vi "VIH Dialog - Compiled HTML Help  Project.vi"(11 "Project Tree":T1) -> ()   [LabVIEW 2014]
doc: "::: VI Helpeks :::\nCopyright (c) 2000-2026 Konstantin Shifershteyn. All rights reserved."
uses:
  VIH Project Tree Typedef - Tree Refnum.ctl
  <vilib>/Platform/browser.llb/Open URL in Default Browser (string).vi
  <vilib>/Platform/browser.llb/Open URL in Default Browser (path).vi
panel:
  in  "Tab Control":enum32{"Project", "Options", "Compile Log"}(tab)
  in  "%HHP New Compile":bool caption="Create & Compile"
  in  "%HHP Info":bool caption="Open Info File"
  in  "%HHP Open":bool caption="Open Project"
  in  "%CHM Open":bool caption="Open CHM File"
  in  "HHP Target Path":path caption="HHP File"
  in  "HHP Target":enum16{"default", "custom"}(ring) caption="Default/Custom selector"
  in  "Default Topic Path":path caption="Default Topic File"
  in  "Default Topic":enum16{"auto", "custom"}(ring) caption="Auto/Custom selector"
  in  "%HHP Explore":bool caption="Explore Folder"
  in  "CHM File Path":path caption="CHM File"
  in  "Custom CHM":enum16{"default", "custom"}(ring) caption="Default/Custom selector"
  in  "Create IDX file":bool=TRUE caption="Generate Index file (HHK)"
  in  "Create TOC file":bool=TRUE caption="Generate Contents file (HHC)"
  in  "%HHP Create":bool caption="Create Project"
  in  "%CHM Compile":bool caption="Create & Compile"
  in  "CHM_AutoBuild":bool caption="Compile CHM file after HTML files are built (HHP file must exist)"
  in  "HHP_AutoBuild":bool caption="Generate HHP file after HTML files are built"
  in  "Open CHM After Compiling":bool=TRUE caption="Open CHM file after compiling"
  in  "HHP Template Path":path caption="HHP Template File"
  in  "HHP Template":enum16{"default", "custom"}(ring) caption="Default/Custom selector"
  in  "OpenAfterBuild":bool=TRUE caption="Open HTML Help Project file (HHP) after creation"
  out "CompileLog":string caption="Compile Log"
  in  "Cancel":bool
  # "*) use Context Help for information on the controls"
  # "HTML Help Project (HHP)"
  # "Compiled Help File (CHM)"
  # "Default Topic (HTML File)"
  # "HHP Template File"
  # "Options used in this utility"
  # "Options used when build from main window"
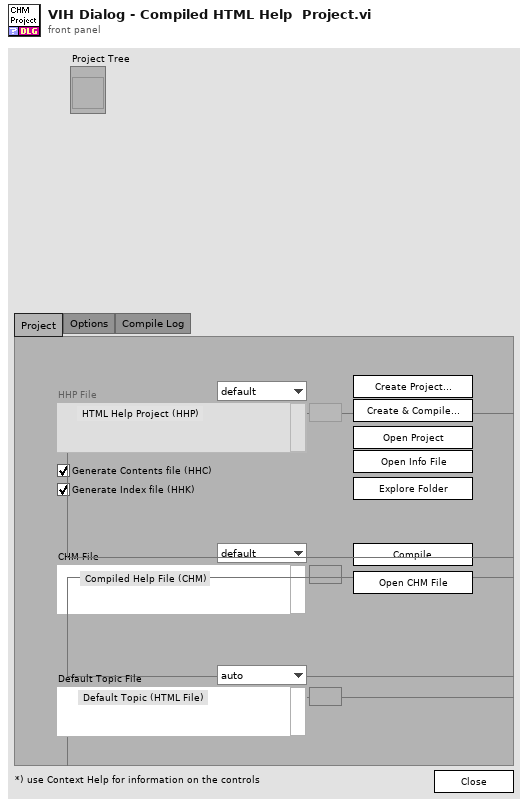
[diagram p1: front panel]
types:
  T1 = typedef "VIH Project Tree Typedef - Tree Refnum.ctl" = refnum<vi>
  T2 = typedef "VIH - CHM Project - HHP Generation Params Cluster.ctl" = cluster{"HHP_Template":enum16{"default", "custom"}, "HHP_Template_CustomPath":path, "HHP_Target":enum16{"default", "custom"}, "HHP_Target_CustomPath":path, "HHP_CreateTOC":bool, "HHP_CreateIDX":bool, "HHP_DefaultTopic":enum16{"auto", "custom"}, "HHP_DefaultTopic_CustomPath":path, "CHM_Filename":path, "HHP_AutoBuild":bool, "CHM_AutoBuild":bool}
  T3 = cluster{"Windows platform":bool, "HHP is associated":bool, "HHC is installed":bool}
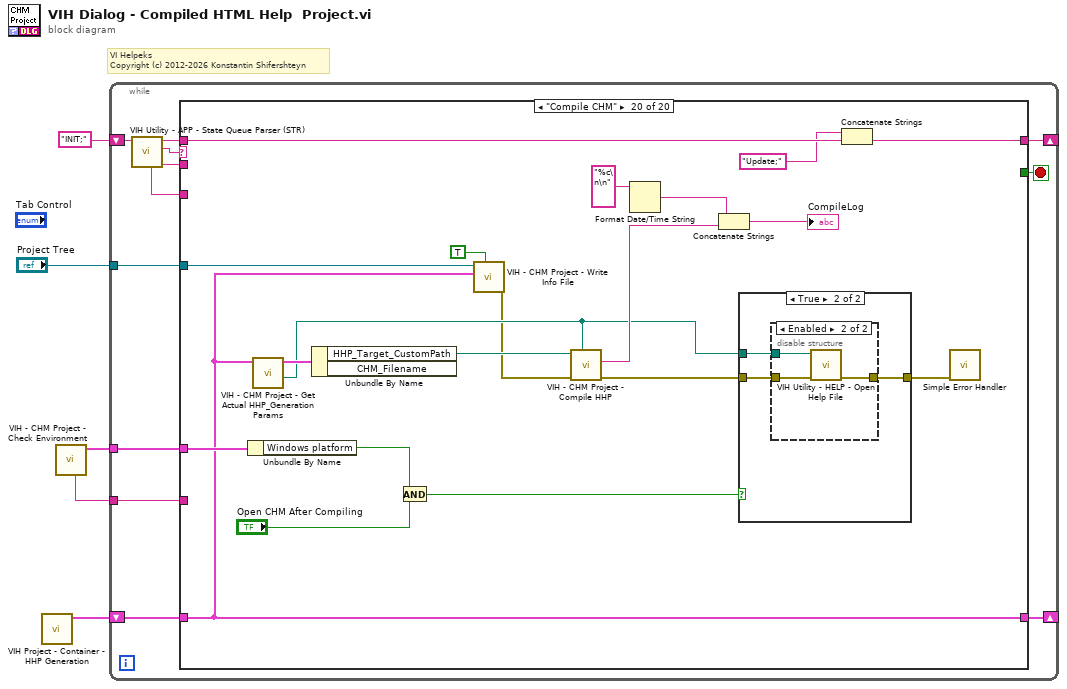
[diagram p0: block diagram]
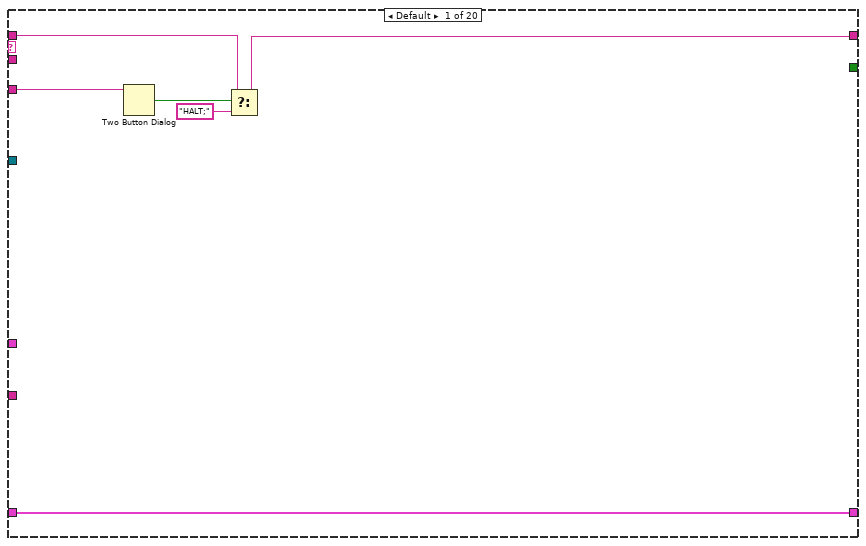
[diagram p2: hidden frame]
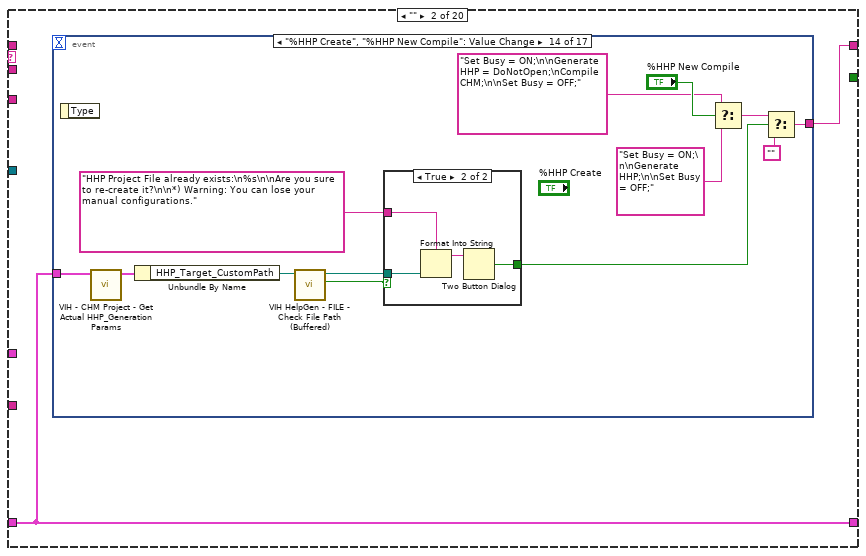
[diagram p3: hidden frame]
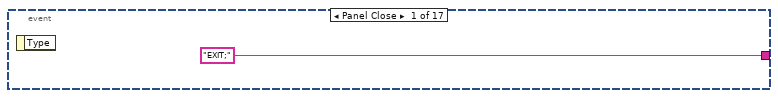
[diagram p4: hidden frame]
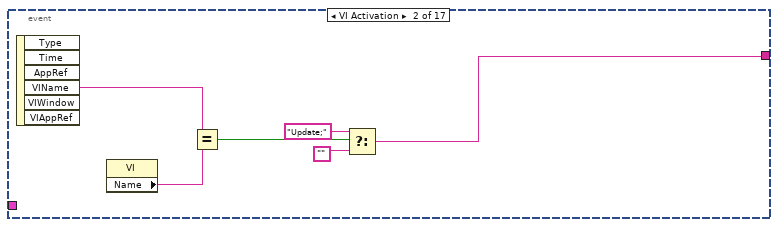
[diagram p5: hidden frame]
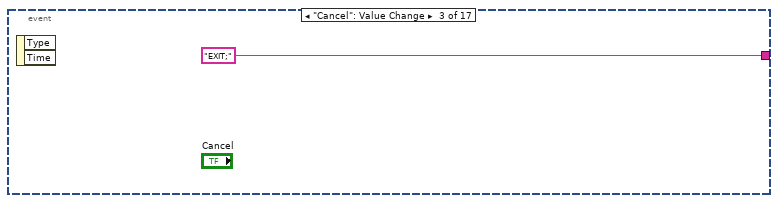
[diagram p6: hidden frame]
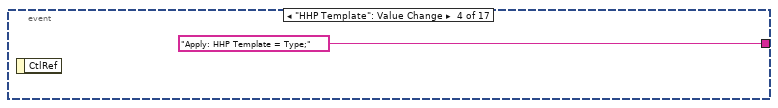
[diagram p7: hidden frame]
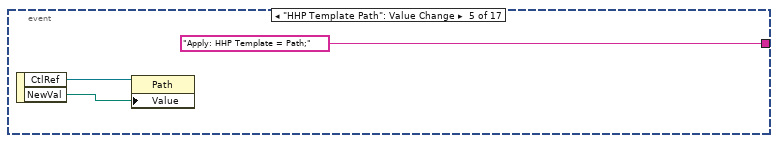
[diagram p8: hidden frame]
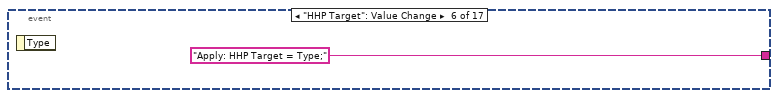
[diagram p9: hidden frame]
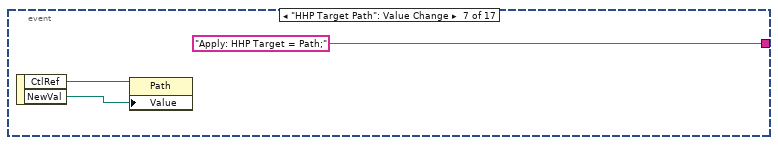
[diagram p10: hidden frame]
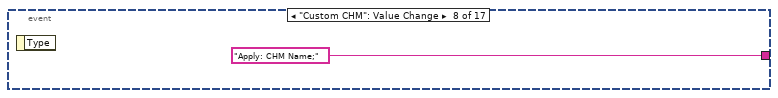
[diagram p11: hidden frame]
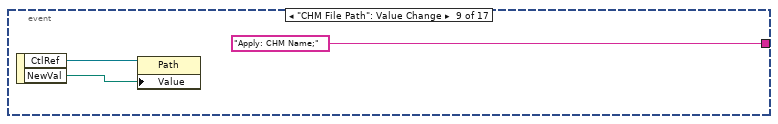
[diagram p12: hidden frame]
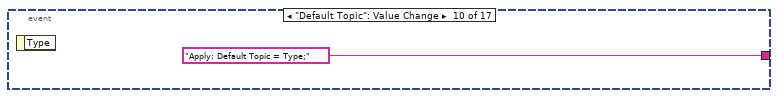
[diagram p13: hidden frame]
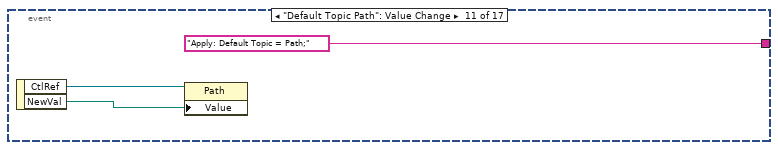
[diagram p14: hidden frame]
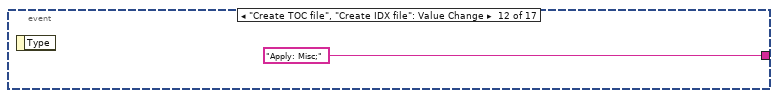
[diagram p15: hidden frame]
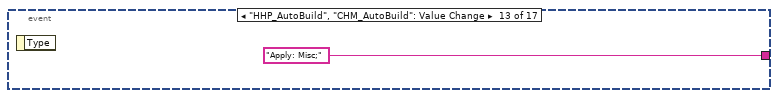
[diagram p16: hidden frame]
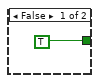
[diagram p17: hidden frame]
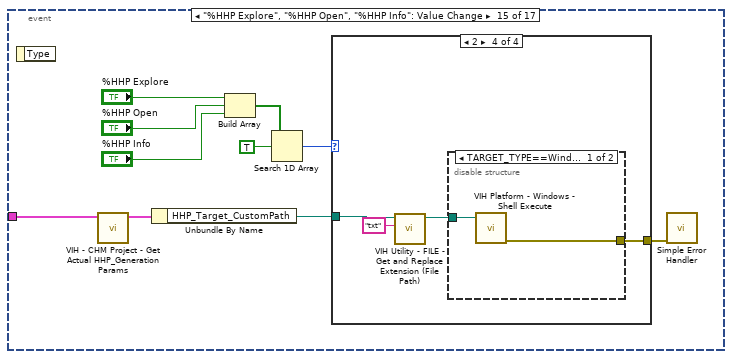
[diagram p18: hidden frame]
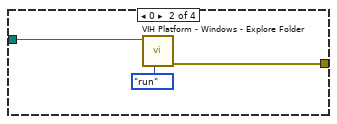
[diagram p20: hidden frame]
diagram:
  # "VI Helpeks\nCopyright (c) 2012-2026 Konstantin Shifershteyn"
  n1 = call "VIH Project - Container - HHP Generation.vi"() -> ("HHP_Generation out"=w4:T2)  [unwired: 11 in]
  n2 = call "VIH - CHM Project - Check Environment.vi"() -> ("Flags"=w2:T3, "Download URL"=w1:string)  [unwired: 8 in, 2 out]
  n3 = while {
    shift-right: [w13] -> _
    shift-left: "INIT;" -> [w17]
    shift-right: [w10] -> _
    shift-left: w4 -> [w9]
    tunnel: "Project Tree" -> [w8]
    tunnel: w2 -> [w7]
    tunnel: w1 -> [w6]
    stop <- w12 stop-if-true
    n4 = call "VIH Utility - APP - State Queue Parser (STR).vi"("input queue"=w17) -> ("state parameters"=w11:string, "state"=w16:string, "remained queue"=w14:string, "complete state specifier"=w15:string)  [unwired: 5 in]
    n5 = case shown="\"Compile CHM\"" w16 {
      tunnel: w15 -> [w23 _ _ _ _ _ _ _ _ _ _ _ _ _ _ _ _ _ _ _]
      tunnel: w14 -> [w21 _ w108 w116 _ w134 w136 w139 w141 w181 w203 w212 w218 w249 w280 w310 w321 w327 w346 w370]
      tunnel: [w20 w25 w107 w116 "HALT;" w134 w136 w139 w141 w167 w201 w212 w217 w248 w279 w309 w320 w327 w339 w367] -> w13
      tunnel: [_ _ _ _ _ TRUE _ _ _ _ _ _ _ _ _ _ _ _ _ _] -> w12
      tunnel: w11 -> [_ _ _ _ w129 _ _ w137 _ _ _ _ w213 w244 w275 _ _ _ w335 _]
      tunnel: [w18 w24 w106 w117 w128 w132 w135 w138 w140 w159 w195 w211 w214 w245 w276 w306 w317 w326 w344 w353] -> w10
      tunnel: w9 -> [w18 w24 w106 w117 w128 w132 w135 w138 w140 w159 w195 w211 w215 w246 w277 w307 w318 w326 w344 w353]
      tunnel: w8 -> [_ _ _ _ _ _ _ _ _ _ _ _ _ _ _ _ _ _ w345 w354]
      tunnel: w7 -> [_ _ w102 w115 _ _ _ _ _ w146 w191 _ _ _ _ _ _ _ w337 w365]
      tunnel: w6 -> [_ _ _ w111 _ _ _ _ _ _ _ _ _ _ _ _ _ _ _ _]
      frame Default {
        n6 = Two Button Dialog(message=w23) -> (T button?=w22:bool)  [unwired: 2 in]
        n7 = Select(t=w21, s=w22, f="HALT;") -> (s? t:f=w20:string)
      }
      frame "" {
        n8 = event shown="[13] \"%HHP Create\", \"%HHP New Compile\": Value Change" {
          selector: _ -> [_ _ _ _ _ _ _ _ _ _ _ _ _ _ _ _ _]
          dyn-events: _ -> [_ _ _ _ _ _ _ _ _ _ _ _ _ _ _ _ _]
          timeout: _ -> [_ _ _ _ _ _ _ _ _ _ _ _ _ _ _ _ _]
          tunnel: ["EXIT;" w27 "EXIT;" "Apply: HHP Template = Type;" "Apply: HHP Template = Path;" "Apply: HHP Target = Type;" "Apply: HHP Target = Path;" "Apply: CHM Name;" "Apply: CHM Name;" "Apply: Default Topic = Type;" "Apply: Default Topic = Path;" "Apply: Misc;" "Apply: Misc;" w55 _ "Set Busy = ON;\n\nCompile CHM;\n\nSet Busy = OFF;" _] -> w25
          tunnel: w24 -> [_ _ _ _ _ _ _ _ _ _ _ _ _ w61 w79 _ w96]
          event Panel Close {
            n9 = event-data() -> ()  [unwired: 1 in, 1 out]
          }
          event VI Activation {
            n10 = event-data() -> ("VIName"=w32:string)  [unwired: 1 in, 5 out]
            n11 = property class="VI"() -> ("Name"=w31:string)  [unwired: 2 in, 2 out]
            n12 = Equal?(x=w32, y=w31) -> (x = y?=w30:bool)
            n13 = Select(t="Update;", s=w30, f="") -> (s? t:f=w27:string)
          }
          event "Cancel": Value Change {
            n14 = event-data() -> ()  [unwired: 1 in, 2 out]
          }
          event "HHP Template": Value Change {
            n15 = event-data() -> ()  [unwired: 1 in, 1 out]
          }
          event "HHP Template Path": Value Change {
            n16 = event-data() -> ("CtlRef"=w36:refnum<vi>, "NewVal"=w35:path)  [unwired: 1 in]
            n17 = property class="Path"(reference=w36, "Value"=w35) -> ()  [unwired: 1 in, 2 out]
          }
          event "HHP Target": Value Change {
            n18 = event-data() -> ()  [unwired: 1 in, 1 out]
          }
          event "HHP Target Path": Value Change {
            n19 = event-data() -> ("CtlRef"=w40:refnum<vi>, "NewVal"=w39:path)  [unwired: 1 in]
            n20 = property class="Path"(reference=w40, "Value"=w39) -> ()  [unwired: 1 in, 2 out]
          }
          event "Custom CHM": Value Change {
            n21 = event-data() -> ()  [unwired: 1 in, 1 out]
          }
          event "CHM File Path": Value Change {
            n22 = event-data() -> ("CtlRef"=w44:refnum<vi>, "NewVal"=w43:path)  [unwired: 1 in]
            n23 = property class="Path"(reference=w44, "Value"=w43) -> ()  [unwired: 1 in, 2 out]
          }
          event "Default Topic": Value Change {
            n24 = event-data() -> ()  [unwired: 1 in, 1 out]
          }
          event "Default Topic Path": Value Change {
            n25 = event-data() -> ("CtlRef"=w48:refnum<vi>, "NewVal"=w47:path)  [unwired: 1 in]
            n26 = property class="Path"(reference=w48, "Value"=w47) -> ()  [unwired: 1 in, 2 out]
          }
          event "Create TOC file", "Create IDX file": Value Change {
            n27 = event-data() -> ()  [unwired: 1 in, 1 out]
          }
          event "HHP_AutoBuild", "CHM_AutoBuild": Value Change {
            n28 = event-data() -> ()  [unwired: 1 in, 1 out]
          }
          event "%HHP Create", "%HHP New Compile": Value Change {
            n29 = event-data() -> ()  [unwired: 1 in, 1 out]
            n30 = call "VIH - CHM Project - Get Actual HHP_Generation Params.vi"("HHP_Generation"=w61) -> ("HHP_Generation out"=w62:T2)  [unwired: 8 in, 2 out]
            n31 = Unbundle By Name(w62) -> ("HHP_Target_CustomPath"=w60:path)
            n32 = call "VIH HelpGen - FILE - Check File Path (Buffered).vi"("File Path"=w60) -> ("Good path"=w59:bool, "dup File Path"=w58:path)  [unwired: 9 in]
            n33 = case shown="True" w59 {
              tunnel: w58 -> [_ w69]
              tunnel: [TRUE w67] -> w57
              tunnel: "HHP Project File already exists:\n%s\n\nAre you sure to re-create it?\n\n*) Warning: You can lose your manual configurations." -> [_ w66]
              frame False {
              }
              frame True {
                n34 = Format Into String(format string=w66, w69) -> (resulting string=w68:string)  [unwired: 2 in, 1 out]
                n35 = Two Button Dialog(message=w68) -> (T button?=w67:bool)  [unwired: 2 in]
              }
            }
            n36 = Select(t="Set Busy = ON;\n\nGenerate HHP = DoNotOpen;\nCompile CHM;\n\nSet Busy = OFF;", s="%HHP New Compile", f="Set Busy = ON;\n\nGenerate HHP;\n\nSet Busy = OFF;") -> (s? t:f=w56:string)
            n37 = Select(t=w56, s=w57, f="") -> (s? t:f=w55:string)
          }
          event "%HHP Explore", "%HHP Open", "%HHP Info": Value Change {
            n38 = event-data() -> ()  [unwired: 1 in, 1 out]
            n39 = call "VIH - CHM Project - Get Actual HHP_Generation Params.vi"("HHP_Generation"=w79) -> ("HHP_Generation out"=w78:T2)  [unwired: 8 in, 2 out]
            n40 = Unbundle By Name(w78) -> ("HHP_Target_CustomPath"=w77:path)
            n41 = Build Array("%HHP Explore", "%HHP Open", "%HHP Info") -> (w72:bool[])
            n42 = Search 1D Array(1D array=w72, element=TRUE) -> (index of element=w70:i32)  [unwired: 1 in]
            n43 = case shown="2" w70 {
              tunnel: w77 -> [_ w82 w84 w87]
              tunnel: [_ w80 w83 w88] -> w76
              frame Default {
              }
              frame 0 {
                n44 = call "VIH Platform - Windows - Explore Folder.vi"("cmd (run)"=enum16{"run", "check"}."run", "exe/doc/dir path"=w82) -> ("error out"=w80:errorcluster)  [unwired: 9 in]
              }
              frame 1 {
                n45 = call "VIH Platform - Windows - Shell Execute.vi"("exe/doc/dir path"=w84) -> ("error out"=w83:errorcluster)  [unwired: 10 in]
              }
              frame 2 {
                n46 = call "VIH Utility - FILE - Get and Replace Extension (File Path).vi"("new extension (none)"="txt", "file path"=w87) -> ("new file path"=w86:path)  [unwired: 8 in, 1 out]
                n47 = disable-structure shown="TARGET_TYPE==Windows" {
                  disable-tunnel: [w90 w91] -> w88
                  disable-tunnel: w86 -> [w89 w92]
                  frame condition #0 (active) {
                    n48 = call "VIH Platform - Windows - Shell Execute.vi"("exe/doc/dir path"=w89) -> ("error out"=w90:errorcluster)  [unwired: 10 in]
                  }
                  frame condition #1 {
                    n49 = call-poly <vilib>:"Open URL in Default Browser.vi"("path"=w92) -> ("error out"=w91:errorcluster)  [unwired: 5 in, 1 out]
                  }
                }
              }
            }
            n50 = call <vilib>:"Simple Error Handler.vi"("error in (no error)"=w76) -> ()  [unwired: 4 in, 5 out]
          }
          event "%CHM Compile": Value Change {
            n51 = event-data() -> ()  [unwired: 1 in, 1 out]
          }
          event "%CHM Open": Value Change {
            n52 = event-data() -> ()  [unwired: 1 in, 1 out]
            n53 = call "VIH - CHM Project - Get Actual HHP_Generation Params.vi"("HHP_Generation"=w96) -> ("CHM File Absolute Path"=w94:path)  [unwired: 8 in, 2 out]
            n54 = call "VIH Utility - HELP - Open Help File.vi"("Help Path"=w94) -> ("error out"=w95:errorcluster)  [unwired: 9 in, 1 out]
            n55 = call <vilib>:"Simple Error Handler.vi"("error in (no error)"=w95) -> ()  [unwired: 4 in, 5 out]
          }
        }
      }
      frame "INIT" {
        n56 = Unbundle By Name(w102) -> ("Windows platform"=w101:bool, "HHP is associated"=w100:bool, "HHC is installed"=w99:bool)
        n57 = call "VIH Utility - UI - Boolean to Control Disable Status.vi"("Status in"=w101) -> ("Control Disable if False"=w104:u8)  [unwired: 3 in, 1 out]
        n58 = call "VIH Utility - UI - Boolean to Control Disable Status.vi"("Status in"=w100) -> ("Control Disable if False"=w103:u8)  [unwired: 3 in, 1 out]
        n59 = call "VIH Utility - UI - Boolean to Control Disable Status.vi"("Status in"=w99) -> ("Control Disable if False"=w98:u8)  [unwired: 3 in, 1 out]
        n60 = local write "CompileLog"("") -> ()
        n61 = property on="%HHP Explore" class="Bool"("DisabledEnum"=w104) -> ()  [unwired: 2 in, 2 out]
        n62 = property on="OpenAfterBuild" class="Bool (strict)"("DisabledEnum"=w103) -> ()  [unwired: 2 in, 2 out]
        n63 = property on="Open CHM After Compiling" class="Bool (strict)"("DisabledEnum"=w98) -> ()  [unwired: 2 in, 2 out]
        n64 = Concatenate Strings("Update;\nINIT Done;" ("string"), w108) -> (w107:string)
        n65 = property on="%HHP New Compile" class="Bool"("DisabledEnum"=w98) -> ()  [unwired: 2 in, 2 out]
      }
      frame "INIT Done" {
        n66 = Unbundle By Name(w115) -> ("Windows platform"=w112:bool, "HHP is associated"=w114:bool)
        n67 = Not(x=w114) -> (.not. x?=w113:bool)
        n68 = First Call?() -> (First Call?: T/F=w110:bool)
        n69 = And(x=w112, y=w113) -> (x .and. y?=w109:bool)
        n70 = And(x=w110, y=w109) -> ()  [unwired: 1 out]
        n71 = case shown="True" w109 {
          tunnel: w111 -> [_ w118]
          frame False {
          }
          frame True {
            n72 = flat-sequence {
              tunnel: "\nMicrosoft HTML Help Workshop is not found.\n\nYou can create HTML Help Project (HHP) with this utility. However, in order to compile a CHM file, you have to install HTML Help Workshop or another program that can process HHP files.\n\nClick the Download button to open HTML Help Workshop download page. Download and run Htmlhelp.exe file and follow the instructions.\n\nNOTE 1: If a message about newer version of HTML Help installed appears during the installation, just ignore it and click OK.\n\nNOTE 2: If this message appears but you already have HTML Help Workshop installed on the computer, make sure HHP file extension is associated with it. Typically, HHP extension is to be associated with HHW.EXE file in either \"C:\\Program Files\\HTML Help Workshop\" or \"C:\\Program Files (x86)\\HTML Help Workshop\" folder.\n" -> [w125]
              tunnel: [w124] -> w119
              frame #0 {
                n73 = call <vilib>:"Beep.vi"() -> ()  [unwired: 12 in]
              }
              frame #1 {
                n74 = Two Button Dialog(message=w125, 1:"Cancel     " ("F button name (\"Cancel\")"), 2:"Download" ("T button name (\"OK\")")) -> (T button?=w124:bool)
              }
            }
            n75 = case shown="True" w119 {
              tunnel: w118 -> [_ w121]
              frame False {
              }
              frame True {
                n76 = call-poly <vilib>:"Open URL in Default Browser.vi"("URL"=w121) -> ()  [unwired: 5 in, 2 out]
              }
            }
          }
        }
      }
      frame "EXIT" {
        w126 = path ""
        n77 = case shown="\"OK\"" w129 {
          tunnel: [_ TRUE] -> _
          frame Default {
          }
          frame "OK" {
          }
        }
        n78 = call "VIH Project - Container - HHP Generation.vi"("cmd (get)"=enum16{"get", "set"}."set", "HHP_Generation in"=w128) -> ()  [unwired: 9 in, 1 out]
        n79 = property on="Default Topic Path" class="Path"("StartPath"=w126) -> ()  [unwired: 2 in, 2 out]
        n80 = property on="CHM File Path" class="Path"("StartPath"=w126) -> ()  [unwired: 2 in, 2 out]
      }
      frame "HALT" {
      }
      frame "---------------------------------- 1" {
      }
      frame "Set Busy" {
        n81 = case shown="\"ON\"" w137 {
          frame Default {
            n82 = call <vilib>:"Unset Busy.vi"() -> ()  [unwired: 11 in, 1 out]
          }
          frame "ON" {
            n83 = call <vilib>:"Set Busy.vi"() -> ()  [unwired: 10 in, 2 out]
          }
        }
      }
      frame "Control Appearance" {
      }
      frame "Update" {
        n84 = call "VIH - CHM Project - Get Actual HHP_Generation Params.vi"("HHP_Generation"=w159) -> ("HHP_Generation out"=w180:T2)  [unwired: 8 in, 2 out]
        n85 = Unbundle By Name(w146) -> ("HHP is associated"=w145:bool)  [unwired: 1 out]
        n86 = Unbundle By Name(w180) -> ("HHP_Template"=w179:enum16{"default", "custom"}, "HHP_Template_CustomPath"=w165:path, "HHP_Target"=w170:enum16{"default", "custom"}, "HHP_Target_CustomPath"=w148:path, "HHP_DefaultTopic"=w169:enum16{"auto", "custom"}, "HHP_DefaultTopic_CustomPath"=w153:path)
        n87 = call "VIH Utility - FILE - Get Path Attributes (Empty-NAP-Rel).vi"("Path"=w153) -> ("Not A Path or Empty path"=w155:bool, "dup Path"=w154:path)  [unwired: 6 in, 3 out]
        n88 = Strip Path(path=w148) -> (stripped path=w152:path)  [unwired: 1 out]
        n89 = Select(t=w152, s=w155, f=w154) -> (s? t:f=w151:path)
        n90 = call "VIH Utility - FILE - Get and Replace Extension (File Path).vi"("new extension (none)"="txt", "file path"=w148) -> ("new file path"=w149:path)  [unwired: 8 in, 1 out]
        n91 = Equal?(x=w170, y=enum16{"default", "custom"}."default") -> (x = y?=w174:bool)
        n92 = Equal?(x=w179, y=enum16{"default", "custom"}."default") -> (x = y?=w177:bool)
        n93 = Equal?(x=w169, y=enum16{"auto", "custom"}."auto") -> (x = y?=w172:bool)
        n94 = call "VIH Utility - UI - Boolean to Control Disable Status.vi"("Status in"=w177) -> ("Control Disable if True"=w176:u8)  [unwired: 3 in, 1 out]
        n95 = call "VIH UI - Test Path.vi"("Path"=w165) -> ("Color"=w163:u32, "dup Path"=w164:path)  [unwired: 7 in, 2 out]
        n96 = call "VIH Utility - UI - Boolean to Control Disable Status.vi"("Status in"=w174) -> ("Control Disable if True"=w175:u8)  [unwired: 3 in, 1 out]
        n97 = call "VIH Utility - UI - Boolean to Control Disable Status.vi"("Status in"=w172) -> ("Control Disable if True"=w171:u8)  [unwired: 3 in, 1 out]
        n98 = call "VIH UI - Test Path.vi"("Ena Empty (F)"=TRUE, "Path"=w153) -> ("Color"=w161:u32, "dup Path"=w162:path)  [unwired: 6 in, 2 out]
        n99 = call "VIH UI - Test Path.vi"("Path"=w148) -> ("Good Path"=w157:bool, "dup Path"=w158:path)  [unwired: 7 in, 2 out]
        n100 = call "VIH UI - Test Path.vi"("Path"=w149) -> ("Good Path"=w143:bool)  [unwired: 7 in, 3 out]
        n101 = And(x=w157, y=w145) -> (x .and. y?=w156:bool)
        n102 = property on="HHP Template" class="Enum (strict)"("Value"=w179) -> ()  [unwired: 2 in, 2 out]
        n103 = property on="HHP Target" class="Enum (strict)"("Value"=w170) -> ()  [unwired: 2 in, 2 out]
        n104 = property on="Default Topic" class="Enum (strict)"("Value"=w169) -> ()  [unwired: 2 in, 2 out]
        n105 = call "VIH Utility - UI - Boolean to Control Disable Status.vi"("Status in"=w156) -> ("Control Disable if False"=w142:u8)  [unwired: 3 in, 1 out]
        n106 = call "VIH Utility - UI - Boolean to Control Disable Status.vi"("Status in"=w143) -> ("Control Disable if False"=w150:u8)  [unwired: 3 in, 1 out]
        n107 = property on="HHP Template Path" class="Path"("DisabledEnum"=w176, "Value"=w164, "Text.TextColor"=w163) -> ()  [unwired: 2 in, 2 out]
        n108 = property on="HHP Target Path" class="Path"("DisabledEnum"=w175, "Value"=w158, "Text.TextColor"=u32 0) -> ()  [unwired: 2 in, 2 out]
        n109 = property on="Default Topic Path" class="Path"("DisabledEnum"=w171, "Value"=w162, "Text.TextColor"=w161, "StartPath"=w151) -> ()  [unwired: 2 in, 2 out]
        n110 = property on="%HHP Open" class="Bool"("DisabledEnum"=w142) -> ()  [unwired: 2 in, 2 out]
        n111 = property on="%HHP Info" class="Bool"("DisabledEnum"=w150) -> ()  [unwired: 2 in, 2 out]
        n112 = Concatenate Strings("Update 2;\nControl Appearance;" ("string"), w181) -> (w167:string)
        n113 = property on="%CHM Compile" class="Bool"("DisabledEnum"=w142) -> ()  [unwired: 2 in, 2 out]
      }
      frame "Update 2" {
        n114 = call "VIH - CHM Project - Get Actual HHP_Generation Params.vi"("HHP_Generation"=w195) -> ("CHM File Absolute Path"=w182:path, "HHP_Generation out"=w202:T2)  [unwired: 8 in, 1 out]
        n115 = Unbundle By Name(w202) -> ("HHP_CreateTOC"=w183:bool, "HHP_CreateIDX"=w184:bool, "CHM_Filename"=w192:path, "HHP_AutoBuild"=w186:bool, "CHM_AutoBuild"=w185:bool)  [unwired: 2 out]
        n116 = Unbundle By Name(w191) -> ("Windows platform"=w190:bool)
        n117 = Unbundle By Name(w195) -> ("CHM_Filename"=w194:path)
        n118 = Empty String/Path?(string/path=w194) -> (empty?=w199:bool)
        n119 = case shown="True" w199 {
          tunnel: [enum16{"default", "custom"}."custom" ("Custom CHM name") enum16{"default", "custom"}."default" ("Custom CHM name")] -> w198
          tunnel: [_ TRUE] -> w197
          frame False {
          }
          frame True {
          }
        }
        n120 = local write "Create TOC file"(w183) -> ()
        n121 = local write "Create IDX file"(w184) -> ()
        n122 = local write "HHP_AutoBuild"(w186) -> ()
        n123 = local write "CHM_AutoBuild"(w185) -> ()
        n124 = call "VIH Utility - UI - Boolean to Control Disable Status.vi"("Status in"=w197) -> ("Control Disable if True"=w196:u8)  [unwired: 3 in, 1 out]
        n125 = disable-structure shown="Enabled" {
          disable-tunnel: [w205 w206] -> w189
          disable-tunnel: w182 -> [w204 w207]
          frame Disabled {
            n126 = call "VIH UI - Test Path.vi"("Path"=w204) -> ("Good Path"=w205:bool)  [unwired: 7 in, 3 out]
          }
          frame Enabled {
            n127 = call "VIH HelpGen - FILE - Check File Path (Buffered).vi"("File Path"=w207) -> ("Good path"=w206:bool)  [unwired: 9 in, 1 out]
          }
        }
        n128 = property on="Custom CHM" class="Enum (strict)"("Value"=w198) -> ()  [unwired: 2 in, 2 out]
        n129 = Strip Path(path=w182) -> (stripped path=w187:path)  [unwired: 1 out]
        n130 = And(x=w190, y=w189) -> ()  [unwired: 1 out]
        n131 = call "VIH Utility - UI - Boolean to Control Disable Status.vi"("Status in"=w189) -> ("Control Disable if False"=w193:u8)  [unwired: 3 in, 1 out]
        n132 = property on="CHM File Path" class="Path"("DisabledEnum"=w196, "Value"=w192, "Text.FontColor"=u32 0, "StartPath"=w187) -> ()  [unwired: 2 in, 2 out]
        n133 = property on="%CHM Open" class="Bool"("DisabledEnum"=w193) -> ()  [unwired: 2 in, 2 out]
        n134 = Concatenate Strings("Control Appearance;" ("string"), w203) -> (w201:string)
      }
      frame "---------------------------------- 2" {
      }
      frame "Apply: HHP Template" {
        n135 = in-place {
          in-place-border: w213 -> [w219]
          n136 = in-place-cluster #1(w215) -> ("HHP_Template"=w224:enum16{"default", "custom"}, "HHP_Template_CustomPath"=w225:path)
          n137 = case shown="\"Type\"" w219 {
            tunnel: [w230 w232 w237] -> w222
            tunnel: w225 -> [_ w232 w236]
            tunnel: [w227 w233 w234] -> w223
            tunnel: w224 -> [w229 w233 _]
            tunnel: "HHP Template Path" -> [w231 _ w235]
            tunnel: "HHP Template" -> [_ _ w234]
            frame "Path" {
              n138 = call "VIH Utility - FILE - Get Path Attributes (Empty-NAP-Rel).vi"("Path"=w231) -> ("Not A Path or Empty path"=w228:bool, "dup Path"=w230:path)  [unwired: 6 in, 3 out]
              n139 = Select(t=enum16{"default", "custom"}."default", s=w228, f=w229) -> (s? t:f=w227:enum16{"default", "custom"})
            }
            frame Default {
            }
            frame "Type" {
              n140 = case shown="\"custom\"" w234 {
                tunnel: [w238 w240] -> w237
                tunnel: w236 -> [w238 w243]
                tunnel: w235 -> [_ w239]
                frame "default" {
                }
                frame "custom" {
                  n141 = call "VIH Utility - FILE - Get Path Attributes (Empty-NAP-Rel).vi"("Path"=w243) -> ("Not A Path or Empty path"=w242:bool, "dup Path"=w241:path)  [unwired: 6 in, 3 out]
                  n142 = Select(t=w239, s=w242, f=w241) -> (s? t:f=w240:path)
                }
              }
            }
          }
          n143 = in-place-cluster #1("HHP_Template"=w223, "HHP_Template_CustomPath"=w222) -> (w214:T2)
        }
        n144 = Concatenate Strings("Update;", w218) -> (w217:string)
      }
      frame "Apply: HHP Target" {
        n145 = in-place {
          in-place-border: w244 -> [w254]
          n146 = in-place-cluster #2(w246) -> ("HHP_Target"=w252:enum16{"default", "custom"}, "HHP_Target_CustomPath"=w255:path)
          n147 = case shown="\"Type\"" w254 {
            tunnel: [w261 w263 w268] -> w256
            tunnel: w255 -> [_ w263 w267]
            tunnel: [w258 w264 w265] -> w253
            tunnel: w252 -> [w260 w264 _]
            tunnel: "HHP Target Path" -> [w262 _ w266]
            tunnel: "HHP Target" -> [_ _ w265]
            frame "Path" {
              n148 = call "VIH Utility - FILE - Get Path Attributes (Empty-NAP-Rel).vi"("Path"=w262) -> ("Not A Path or Empty path"=w259:bool, "dup Path"=w261:path)  [unwired: 6 in, 3 out]
              n149 = Select(t=enum16{"default", "custom"}."default", s=w259, f=w260) -> (s? t:f=w258:enum16{"default", "custom"})
            }
            frame Default {
            }
            frame "Type" {
              n150 = case shown="\"custom\"" w265 {
                tunnel: [w269 w271] -> w268
                tunnel: w267 -> [w269 w274]
                tunnel: w266 -> [_ w270]
                frame "default" {
                }
                frame "custom" {
                  n151 = call "VIH Utility - FILE - Get Path Attributes (Empty-NAP-Rel).vi"("Path"=w274) -> ("Not A Path or Empty path"=w273:bool, "dup Path"=w272:path)  [unwired: 6 in, 3 out]
                  n152 = Select(t=w270, s=w273, f=w272) -> (s? t:f=w271:path)
                }
              }
            }
          }
          n153 = in-place-cluster #2("HHP_Target"=w253, "HHP_Target_CustomPath"=w256) -> (w245:T2)
        }
        n154 = Concatenate Strings("Update;", w249) -> (w248:string)
      }
      frame "Apply: Default Topic" {
        n155 = in-place {
          in-place-border: w275 -> [w285]
          n156 = in-place-cluster #3(w277) -> ("HHP_DefaultTopic"=w283:enum16{"auto", "custom"}, "HHP_DefaultTopic_CustomPath"=w286:path)
          n157 = case shown="\"Type\"" w285 {
            tunnel: [w292 w294 w299] -> w287
            tunnel: w286 -> [_ w294 w298]
            tunnel: [w289 w295 w296] -> w284
            tunnel: w283 -> [w291 w295 _]
            tunnel: "Default Topic Path" -> [w293 _ w297]
            tunnel: "Default Topic" -> [_ _ w296]
            frame "Path" {
              n158 = call "VIH Utility - FILE - Get Path Attributes (Empty-NAP-Rel).vi"("Path"=w293) -> ("Not A Path or Empty path"=w290:bool, "dup Path"=w292:path)  [unwired: 6 in, 3 out]
              n159 = Select(t=enum16{"auto", "custom"}."auto", s=w290, f=w291) -> (s? t:f=w289:enum16{"auto", "custom"})
            }
            frame Default {
            }
            frame "Type" {
              n160 = case shown="\"custom\"" w296 {
                tunnel: [w300 w302] -> w299
                tunnel: w298 -> [w300 w305]
                tunnel: w297 -> [_ w301]
                frame "auto" {
                }
                frame "custom" {
                  n161 = call "VIH Utility - FILE - Get Path Attributes (Empty-NAP-Rel).vi"("Path"=w305) -> ("Not A Path or Empty path"=w304:bool, "dup Path"=w303:path)  [unwired: 6 in, 3 out]
                  n162 = Select(t=w301, s=w304, f=w303) -> (s? t:f=w302:path)
                }
              }
            }
          }
          n163 = in-place-cluster #3("HHP_DefaultTopic"=w284, "HHP_DefaultTopic_CustomPath"=w287) -> (w276:T2)
        }
        n164 = Concatenate Strings("Update;", w280) -> (w279:string)
      }
      frame "Apply: CHM Name" {
        n165 = in-place {
          n166 = in-place-cluster #4(w307) -> ()  [unwired: 1 out]
          n167 = Equal?(x="Custom CHM", y=enum16{"default", "custom"}."default") -> (x = y?=w314:bool)
          n168 = Select(t=path "", s=w314, f="CHM File Path") -> (s? t:f=w312:path)
          n169 = in-place-cluster #4("CHM_Filename"=w312) -> (w306:T2)
        }
        n170 = Concatenate Strings("Update;", w310) -> (w309:string)
      }
      frame "Apply: Misc" {
        n171 = in-place {
          n172 = in-place-cluster #5(w318) -> ()  [unwired: 4 out]
          n173 = in-place-cluster #5("HHP_CreateTOC"="Create TOC file", "HHP_CreateIDX"="Create IDX file", "HHP_AutoBuild"="HHP_AutoBuild", "CHM_AutoBuild"="CHM_AutoBuild") -> (w317:T2)
        }
        n174 = Concatenate Strings("Update;", w321) -> (w320:string)
      }
      frame "---------------------------------- 3" {
      }
      frame "Generate HHP" {
        n175 = Unbundle By Name(w337) -> ("HHP is associated"=w336:bool)
        n176 = To Lower Case(string=w335) -> (all lower case string=w334:string)
        n177 = To Lower Case(string="DoNotOpen" ("y")) -> (all lower case string=w332:string)
        n178 = Not Equal?(x=w334, y=w332) -> (x != y?=w329:bool)
        n179 = call "VIH - CHM Project - Create Project Files.vi"("HHP_Generation"=w344, "Project Tree"=w345) -> ("error out"=w342:errorcluster, "Target HHP File"=w341:path)  [unwired: 7 in, 1 out]
        n180 = And(x="OpenAfterBuild", y=w336) -> (x .and. y?=w331:bool)
        n181 = And(x=w329, y=w331) -> (x .and. y?=w330:bool)
        n182 = case shown="True" w330 {
          tunnel: w342 -> [w347 w350]
          tunnel: [w347 w349] -> w343
          tunnel: w341 -> [_ w348]
          frame False {
          }
          frame True {
            n183 = call "VIH Platform - Windows - Shell Execute.vi"("error in"=w350, "exe/doc/dir path"=w348) -> ("error out"=w349:errorcluster)  [unwired: 9 in]
          }
        }
        n184 = local write "CompileLog"("") -> ()
        n185 = call <vilib>:"Simple Error Handler.vi"("error in (no error)"=w343) -> ()  [unwired: 4 in, 5 out]
        n186 = Concatenate Strings("Update;" ("string"), w346) -> (w339:string)
      }
      frame "Compile CHM" {
        n187 = Unbundle By Name(w365) -> ("Windows platform"=w364:bool)
        n188 = call "VIH - CHM Project - Get Actual HHP_Generation Params.vi"("HHP_Generation"=w353) -> ("CHM File Absolute Path"=w355:path, "HHP_Generation out"=w362:T2)  [unwired: 8 in, 1 out]
        n189 = Unbundle By Name(w362) -> ("HHP_Target_CustomPath"=w361:path)  [unwired: 1 out]
        n190 = And(x="Open CHM After Compiling", y=w364) -> (x .and. y?=w368:bool)
        n191 = call "VIH - CHM Project - Write Info File.vi"("Expect HHP exist (T)"=TRUE, "HHP_Generation"=w353, "Project Tree"=w354) -> ("error out"=w352:errorcluster)  [unwired: 5 in, 3 out]
        n192 = call "VIH - CHM Project - Compile HHP.vi"("CHM File Path"=w355, "error in"=w352, "HHP File Path"=w361) -> ("error out"=w360:errorcluster, "Log"=w359:string)  [unwired: 6 in, 1 out]
        n193 = Format Date/Time String(time format string (%c)="%c\n\n") -> (date/time string=w357:string)  [unwired: 2 in]
        n194 = Concatenate Strings(w357, w359) -> (→"CompileLog":string)
        n195 = case shown="True" w368 {
          tunnel: w360 -> [w371 w374]
          tunnel: [w371 w373] -> w369
          tunnel: w355 -> [_ w372]
          frame False {
          }
          frame True {
            n196 = disable-structure shown="Enabled" {
              disable-tunnel: w374 -> [w377 w379]
              disable-tunnel: [w376 w378] -> w373
              disable-tunnel: w372 -> [w375 w380]
              frame Disabled {
                n197 = call "VIH Platform - Windows - Shell Execute.vi"("error in"=w377, "exe/doc/dir path"=w375) -> ("error out"=w376:errorcluster)  [unwired: 9 in]
              }
              frame Enabled {
                n198 = call "VIH Utility - HELP - Open Help File.vi"("error in"=w379, "Help Path"=w380) -> ("error out"=w378:errorcluster)  [unwired: 8 in, 1 out]
              }
            }
          }
        }
        n199 = Concatenate Strings("Update;" ("string"), w370) -> (w367:string)
        n200 = call <vilib>:"Simple Error Handler.vi"("error in (no error)"=w369) -> ()  [unwired: 4 in, 5 out]
      }
    }
  }
